vi "Write.vi"(8 "error in (no error)":errorcluster, 10 "Boolean":bool, 11 "Boolean in":refnum<class "CTI_GPIO_DigitalOut.lvclass">) -> (0 "error out":errorcluster, 3 "Boolean out":refnum<class "CTI_GPIO_DigitalOut.lvclass">)   [LabVIEW 2021, in "CTI_GPIO_DigitalOut.lvclass"]
doc: "Abstract Data Classes 2.1.1.13\nTim Streeter - TSA\nCopyright (c) 2025, TSA"
uses:
  CTI_GPIO_DigitalOut.lvclass
  CTI_GPIO_DigitalOut.lvclass/CTI_GPIO_DigitalOut.ctl
  <vilib>/CTI/CTI Drivers/CTI/Session/Session.lvclass
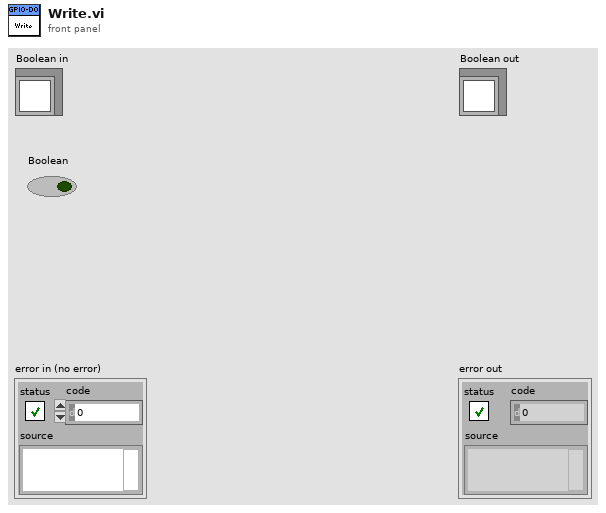
[diagram p1: front panel]
types:
  T1 = typedef "CTI.lvlib/GPIO Number.ctl" = i8
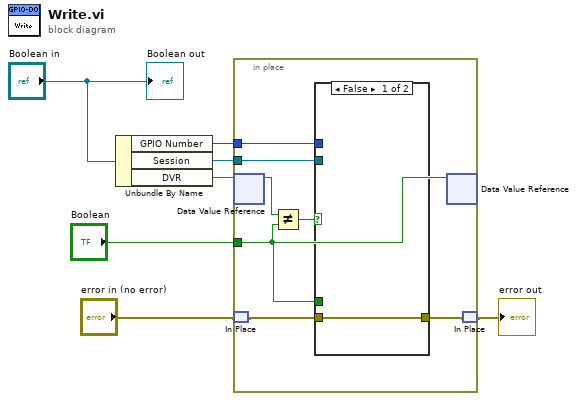
[diagram p0: block diagram]
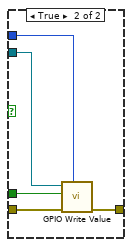
[diagram p2: hidden frame]
diagram:
  n1 = Unbundle By Name("Boolean in") -> ("GPIO Number"=w5:T1, "Session"=w4:refnum<class "Session.lvclass">, "DVR"=w3:refnum<data-value>)
  n2 = in-place {
    in-place-border: "Boolean" -> [w12]
    in-place-border: w5 -> [w14]
    in-place-border: w4 -> [w13]
    n3 = in-place-dvr #1(w3) -> (w11:bool)  [unwired: 1 out]
    n4 = in-place-match #2("error in (no error)") -> (w10:errorcluster)
    n5 = Not Equal?(x=w11, y=w12) -> (x != y?=w8:bool)
    n6 = case shown="False" w8 {
      tunnel: w14 -> [_ w20]
      tunnel: w13 -> [_ w19]
      tunnel: w12 -> [_ w18]
      tunnel: w10 -> [w15 w17]
      tunnel: [w15 w16] -> w9
      frame False {
      }
      frame True {
        n7 = call <vilib>:"GPIO Write Value.vi"("GPIO #"=w20, "error in (no error)"=w17, "Value"=w18, "Session in"=w19) -> ("error out"=w16:errorcluster)  [unwired: 6 in, 1 out]
      }
    }
    n8 = in-place-dvr #1(w12) -> ()  [unwired: 2 out]
    n9 = in-place-match #2(w9) -> (→"error out":errorcluster)
  }
  "Boolean out" <- "Boolean in"
